vi "Create Boolean Channels.vi"(6 "Input?":bool, 8 "error in (no error)":errorcluster, 9 "New Number of Channels":i32, 10 "Boolean Channels in":T1[](array[typedef]), 11 "Modbus in":refnum<class "Modbus.lvclass">) -> (0 "error out":errorcluster, 1 "Channels to remove":string[](array[string]), 2 "Boolean channels out":T1[](array[typedef]), 3 "Modbus out":refnum<class "Modbus.lvclass">)   [LabVIEW 2026, in "Modbus.lvlib" / "Modbus.lvclass"]
uses:
  Modbus.lvclass
  Types/Boolean Data.ctl
  Types/Modbus Table.ctl
  <vilib>/FlexLogger/SDK/PluginSDK.lvlibp/PEFClasses/SDK/Channel/Channel.lvclass
  C:/Program Files/National Instruments/LabVIEW 2026/vi.lib/FlexLogger/SDK/PluginSDK.lvlibp/PEFClasses/SDK/Plugin/Plugin.lvclass
  <vilib>/FlexLogger/SDK/PluginSDK.lvlibp/PEFClasses/SDK/Plugin/Plugin.lvclass
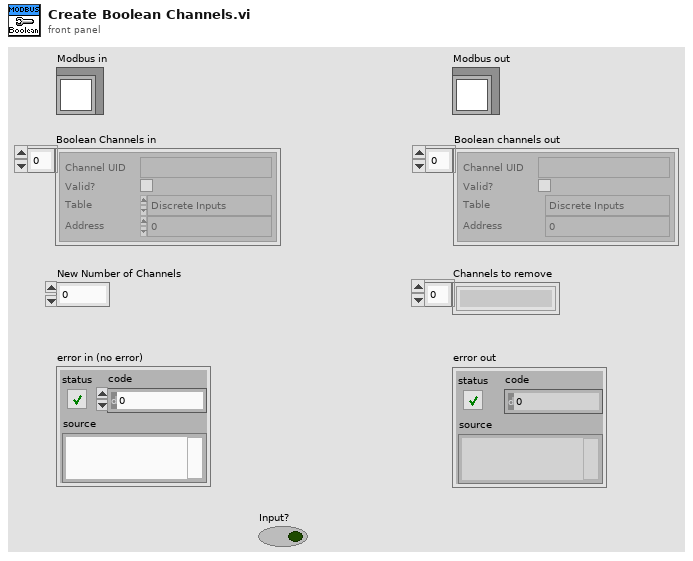
[diagram p1: front panel]
types:
  T1 = typedef "Modbus.lvlib/Modbus.lvclass/Boolean Data.ctl" = cluster{"Channel UID":string, "Valid?":bool, "Table":T2, "Address":i32}
  T2 = typedef "Modbus.lvlib/Modbus.lvclass/Modbus Table.ctl" = enum16{"Discrete Inputs", "Coils", "Input Registers", "Holding Registers"}
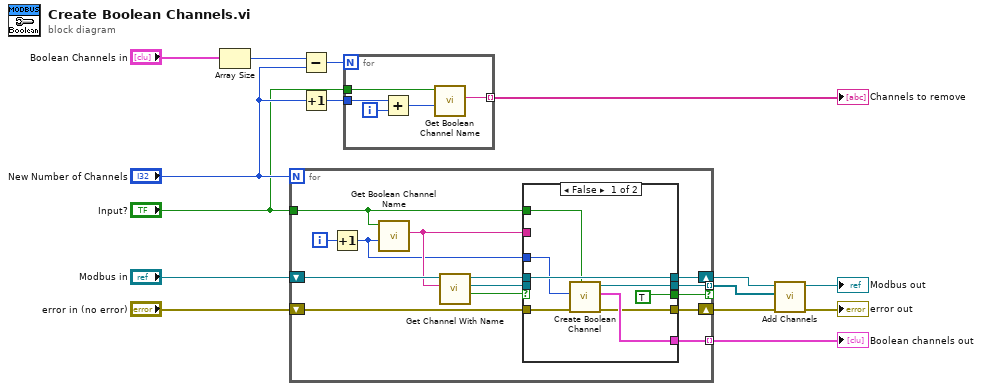
[diagram p0: block diagram]
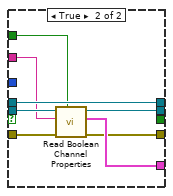
[diagram p2: hidden frame]
diagram:
  n1 = Array Size(array="Boolean Channels in") -> (size(s)=w4:i32)
  n2 = for {
    N: "New Number of Channels" -> [_]
    tunnel: [w27] -> w8 mode=indexing if=w26
    shift-right: [w25] -> w9
    shift-left: "error in (no error)" -> [w24]
    shift-right: [w19] -> w7
    shift-left: "Modbus in" -> [w29]
    tunnel: [w23] -> w10 mode=indexing
    tunnel: "Input?" -> [w16]
    i -> [w22]
    n3 = Increment(x=w22) -> (x+1=w17:i32)
    n4 = call "Get Boolean Channel Name.vi"("Channel Numer"=w17, "Input?"=w16) -> ("Bool Channel ID"=w28:string)  [unwired: 8 in, 1 out]
    n5 = call <vilib>:"Get Channel With Name.vi"("Name"=w28, "Plugin in"=w29) -> ("Found?"=w18:bool, "Channel"=w21:refnum<class "Channel.lvclass">, "Plugin out"=w20:refnum<class "Modbus.lvclass">)  [unwired: 7 in]
    n6 = case shown="False" w18 {
      tunnel: w28 -> [_ w39]
      tunnel: [w33 w41] -> w27
      tunnel: [TRUE _] -> w26
      tunnel: [w32 w40] -> w25
      tunnel: w24 -> [w36 w44]
      tunnel: [w35 w43] -> w23
      tunnel: w21 -> [_ w45]
      tunnel: w20 -> [w34 w42]
      tunnel: [w34 w42] -> w19
      tunnel: w16 -> [w30 w38]
      tunnel: w17 -> [w31 _]
      frame False {
        n7 = call "Create Boolean Channel.vi"("Input?"=w30, "error in (no error)"=w36, "Channel Number"=w31) -> ("error out"=w32:errorcluster, "Boolean Channel"=w35:T1, "Channel out"=w33:refnum<class "Channel.lvclass">)  [unwired: 6 in]
      }
      frame True {
        n8 = call "Read Boolean Channel Properties.vi"("Input?"=w38, "error in (no error)"=w44, "Bool Channel ID"=w39, "Channel in"=w45) -> ("error out"=w40:errorcluster, "Boolean Channel"=w43:T1, "Channel out"=w41:refnum<class "Channel.lvclass">)  [unwired: 5 in]
      }
    }
  }
  "Boolean channels out" <- w10
  n9 = Subtract(x=w4, y="New Number of Channels") -> (x-y=w3:i32)
  n10 = Increment(x="New Number of Channels") -> (x+1=w2:i32)
  n11 = for {
    N: w3 -> [_]
    tunnel: [w47] -> w13 mode=indexing
    tunnel: w2 -> [w49]
    tunnel: "Input?" -> [w48]
    i -> [w50]
    n12 = Add(x=w49, y=w50) -> (x+y=w46:i32)
    n13 = call "Get Boolean Channel Name.vi"("Channel Numer"=w46, "Input?"=w48) -> ("Bool Channel ID"=w47:string)  [unwired: 8 in, 1 out]
  }
  "Channels to remove" <- w13
  n14 = call <vilib>:"Add Channels.vi"("error in (no error)"=w9, "Channels"=w8, "Plugin in"=w7) -> ("error out"=→"error out":errorcluster, "Plugin out"=→"Modbus out":refnum<class "Modbus.lvclass">)  [unwired: 7 in]
